vi "Earth Detection.vi"(6 "error in":errorcluster) -> (0 "error out":errorcluster, 1 "Command Response":string, 2 "Measured Data":string, 3 "number":dbl)   [LabVIEW 2021]
uses:
  DUT/DUT_Cmd.ctl
panel:
  out "Result":string
  out "RESULT":bool
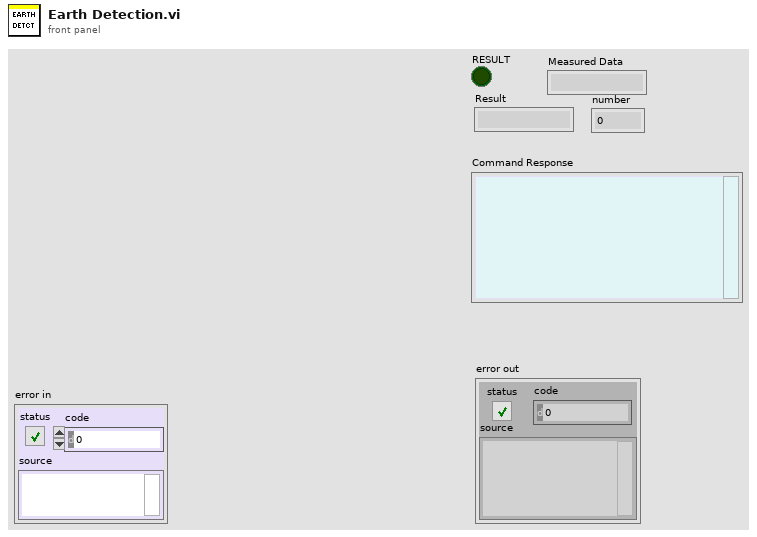
[diagram p1: front panel]
types:
  T1 = typedef "DUT_Cmd.ctl" = enum16{"Unlock serial", "Stop console logs", "Release emergency at start", "Read firmware", "WiFi credentials", "WiFi connected", "WiFi SSID", "Board revision", "ADC_NTC_TEMP", "ADC_TYPE2_RCD_CURRENT", "PCBA serial write", "PCBA serial readback", "Start energy meter", "Energy meter Vac", "Energy meter Iac", "Energy meter PF", "Energy meter energy", "Provision", "Set gateway identity", "CP checklist", "Earth detect", "D+M sense unplugged", "D+M sense plugged", "Output relay weld", "Start diagnostics", "Relay 1 on", "Relay 2 on", "Emergency pressed", "Release emergency", "Emergency released", "Unlock serial for 5 A", "Board current (5 A)", "Unlock serial for 15 A", "Board current (15 A)", "Unlock serial for 0 A", "NFC tag", "Start diagnostics again", "Relay 2 off", "Relay 1 off", "End diagnostics", "Load current (5 A) [No USB station]", "Load current (15 A) [No USB station]", "Load current (0 A) [No USB station]", "NFC tag [No USB station]", "Battery Voltage", "FW Power reset", "Notification LED", "O/P Relay weld Detection", "Earth Detection", "12V ", "5V", "3.3V", "Reboot"}
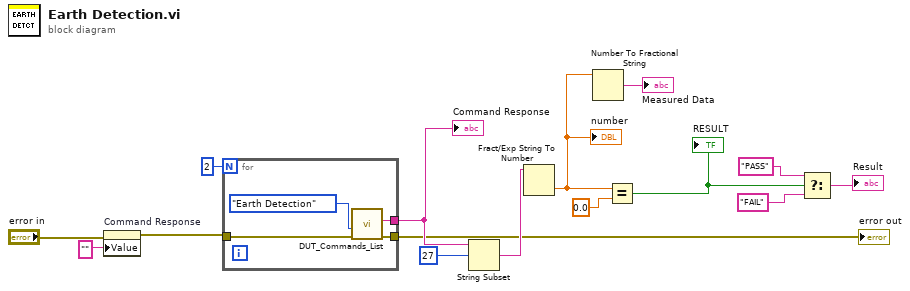
[diagram p0: block diagram]
diagram:
  n1 = property on="Command Response" class="Str"(error in="error in", "Value"="" ("Command Response")) -> (error out=w11:errorcluster)  [unwired: 1 in, 1 out]
  n2 = for {
    N: 2 -> [_]
    tunnel: [w17] -> w9
    tunnel: w11 -> [w18]
    tunnel: [w16] -> w4
    n3 = call "DUT_Commands_List.vi"("error in"=w18, "DUT Cmd"=DUT_Cmd."Earth Detection") -> ("error out"=w16:errorcluster, "Command Response"=w17:string)  [unwired: 7 in, 1 out]
  }
  "error out" <- w4
  "Command Response" <- w9
  n4 = String Subset(string=w9, offset (0)=27) -> (substring=w7:string)  [unwired: 1 in]
  n5 = Fract/Exp String To Number(string=w7) -> (number=w2:dbl)  [unwired: 3 in, 1 out]
  "number" <- w2
  n6 = Number To Fractional String(number=w2) -> (F-format string=→"Measured Data":string)  [unwired: 3 in]
  n7 = Equal?(x=w2, y=0.0 ("lower limit")) -> (x = y?=w5:bool)
  "RESULT" <- w5
  n8 = Select(t="PASS", s=w5, f="FAIL") -> (s? t:f=→"Result":string)
